vi "Stop.vi"(8 "error in (no error)":errorcluster, 11 "CAN RW CANsub in":refnum<class "CAN RW CANsub.lvclass">) -> (0 "error out":errorcluster, 3 "CAN RW CANsub out":refnum<class "CAN RW CANsub.lvclass">)   [LabVIEW 2021, in "CAN RW CANsub.lvclass"]
uses:
  CAN RW CANsub.lvclass
  CAN RW CANsub.lvclass/CAN RW CANsub.ctl
  CANsub/c_client/api/CANsub_Channel/CANsub_Channel.lvclass
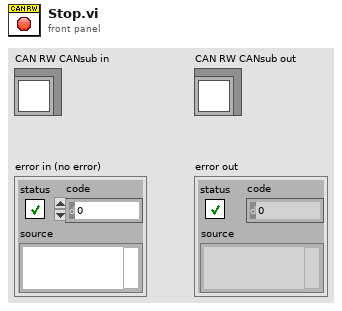
[diagram p1: front panel]
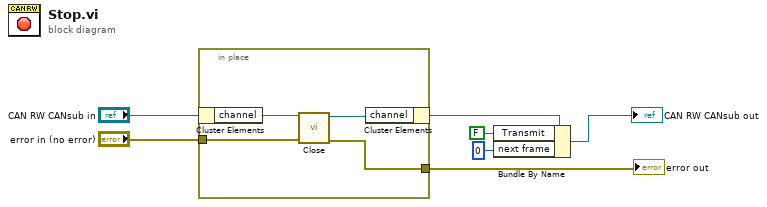
[diagram p0: block diagram]
diagram:
  n1 = in-place {
    in-place-border: "error in (no error)" -> [w10]
    in-place-border: [w8] -> w1
    n2 = in-place-cluster #1("CAN RW CANsub in") -> ("channel"=w11:refnum<class "CANsub_Channel.lvclass">)
    n3 = call-dynamic "Close.vi"("error in (no error)"=w10, "channel in"=w11) -> ("error out"=w8:errorcluster, "channel out"=w9:refnum<class "CANsub_Channel.lvclass">)  [unwired: 8 in]
    n4 = in-place-cluster #1("channel"=w9) -> (w5:refnum<class "CAN RW CANsub.lvclass">)
  }
  "error out" <- w1
  n5 = Bundle By Name(cluster=w5, "Transmit"=FALSE, "next frame"=0) -> (→"CAN RW CANsub out":refnum<class "CAN RW CANsub.lvclass">)
